vi "Init_SV.vi"(8 "error in":errorcluster) -> (0 "error out":errorcluster)   [LabVIEW 2025]
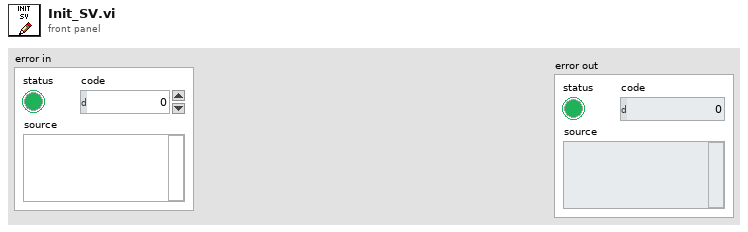
[diagram p1: front panel]
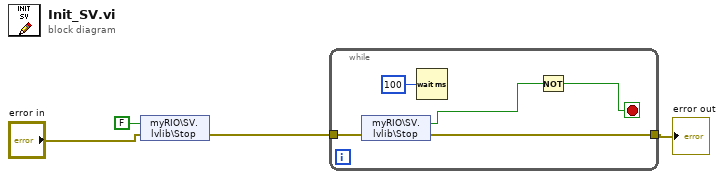
[diagram p0: block diagram]
diagram:
  n1 = shared-variable "myRIO\\SV.lvlib\\Stop"(FALSE ("Stop"), error in="error in") -> (error out=w2:errorcluster)
  n2 = while {
    tunnel: w2 -> [w9]
    tunnel: [w5] -> w1
    stop <- w6 stop-if-true
    n3 = shared-variable "myRIO\\SV.lvlib\\Stop"(error in=w9) -> (w8:bool, error out=w5:errorcluster)
    n4 = Wait (ms)(milliseconds to wait=u32 100) -> ()  [unwired: 1 out]
    n5 = Not(x=w8) -> (.not. x?=w6:bool)
  }
  "error out" <- w1
